vi "matrixreadnumber.vi"(8 "順前削減配列Max no マトリクス":i32[](array[numeric]), 11 "順前削減配列 Max L マトリクス":string[](array[string])) -> (0 "2以上ある?":bool, 1 "MAXリード数":i32, 2 "MAXリード数昇順":i32[](array[numeric]), 3 "Lリード配列昇順":string[](array[string]), 4 "MAXリード":string)   [LabVIEW 2018]
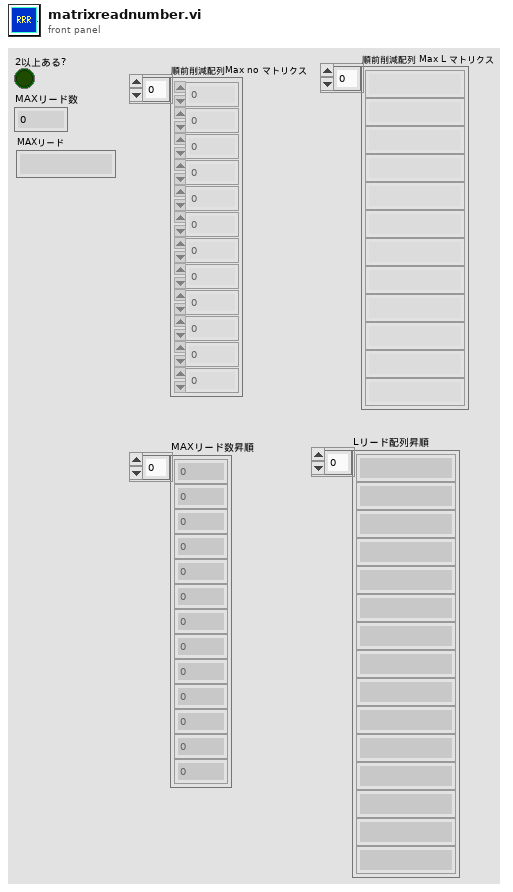
[diagram p1: front panel]
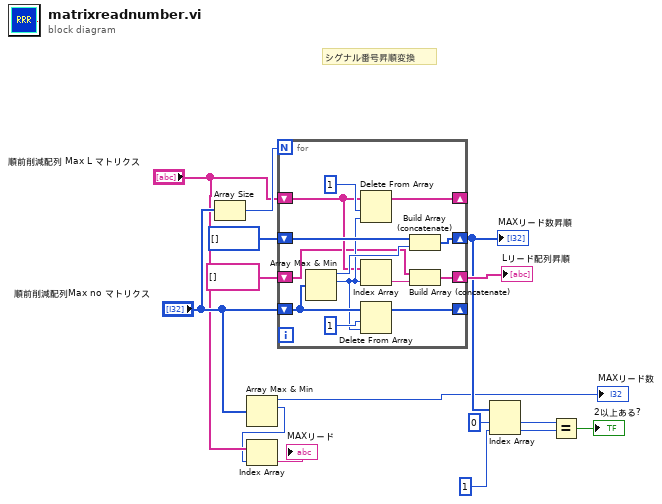
[diagram p0: block diagram]
diagram:
  # "シグナル番号昇順変換"
  n1 = Array Size(array="順前削減配列Max no マトリクス") -> (size(s)=w15:i32)
  n2 = Array Max & Min(array="順前削減配列Max no マトリクス") -> (max value=→"MAXリード数":i32, max index (indices)=w2:i32)  [unwired: 2 out]
  n3 = Index Array(array="順前削減配列 Max L マトリクス", index=w2) -> (element=→"MAXリード":string)
  n4 = for {
    N: w15 -> [_]
    shift-right: [w27] -> _
    shift-left: "順前削減配列Max no マトリクス" -> [w26]
    shift-right: [w24] -> w10
    shift-left: i32[] [] -> [w23]
    shift-right: [w20] -> _
    shift-left: "順前削減配列 Max L マトリクス" -> [w19]
    shift-right: [w17] -> w12
    shift-left: string[] [] -> [w16]
    n5 = Array Max & Min(array=w26) -> (max value=w25:i32, max index (indices)=w21:i32)  [unwired: 2 out]
    n6 = Delete From Array(array=w19, length=1 ("長さ"), index=w21) -> (array with subset deleted=w20:string[])  [unwired: 1 out]
    n7 = Index Array(array=w19, index=w21) -> (element=w18:string)
    n8 = Delete From Array(array=w26, length=1 ("長さ"), index=w21) -> (array with subset deleted=w27:i32[])  [unwired: 1 out]
    n9 = Build Array (concatenate)(w23, w25) -> (w24:i32[])
    n10 = Build Array (concatenate)(w16, w18) -> (w17:string[])
  }
  "Lリード配列昇順" <- w12
  "MAXリード数昇順" <- w10
  n11 = Index Array(array=w10, index #1=0 ("指標"), index #2=1 ("指標")) -> (element #1=w8:i32, element #2=w7:i32)
  n12 = Equal?(x=w8, y=w7) -> (x = y?=→"2以上ある?":bool)
